vi "XPN Copy Latest Frame To Image.vi"(8 "error in (no error)":errorcluster, 10 "LVLineWidthPixels":i32, 11 "LVImagePtr":u64) -> (0 "error out":errorcluster, 3 "function return":i32)   [LabVIEW 2022 SP3, in "xPanelWrapper.lvlib"]
doc: "XPN_API int XPN_CopyLatestFrameToImage(uint64_t LVImagePtr,\n int LVLineWidthPixels);"
uses:
  xPanelWrapper.lvlib
  xPanelWrapper.dll
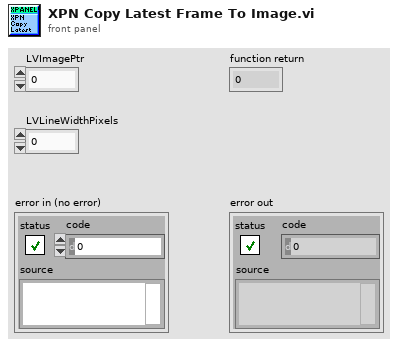
[diagram p1: front panel]
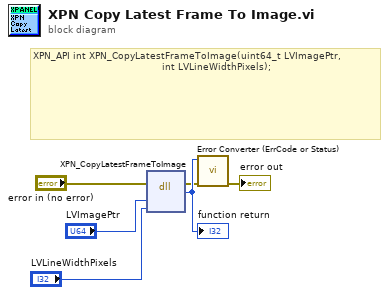
[diagram p0: block diagram]
diagram:
  # "XPN_API int XPN_CopyLatestFrameToImage(uint64_t LVImagePtr,\n                                           int LVLineWidthPixels);"
  n1 = dll-call lib="E:/SourceCodes/image-harvest/ImageHandler/xPanelWrapperLvLib/xPanelWrapper.*" fn="XPN_CopyLatestFrameToImage"(error in="error in (no error)", "LVImagePtr"="LVImagePtr", "LVLineWidthPixels"="LVLineWidthPixels") -> (error out=w2:errorcluster, w6:i32)  [unwired: 4 in, 1 out]
  "function return" <- w6
  n2 = call "Error Converter (ErrCode or Status).vi"("error in (no error)"=w2, "error code"=w6) -> ("error out"=→"error out":errorcluster)  [unwired: 9 in]
